vi "GearCollecter_OperatorAssist.vi"(6 "CatchPosition":dbl, 7 "ReturnToCatch":bool, 8 "CarriageReturned":bool, 9 "Manual_Overide":bool, 10 "Start":bool, 11 "Gear_Beam_Break_Sensor_Triggered":bool) -> (0 "Gear_Rail_Position":dbl, 1 "GearChuteExtend":bool, 2 "Catch_Complete?":bool, 3 "Gate_Pos":T1, 4 "Current_State":T2)   [LabVIEW 2016]
uses:
  TypeDefs/GearCollectState_Type.ctl
  TypeDefs/GatePos_Type.ctl
  ArgosLib/Signal Processing/TypeDefs/EdgeDetector_Type.ctl
  ArgosLib/ArgosLib.lvlib
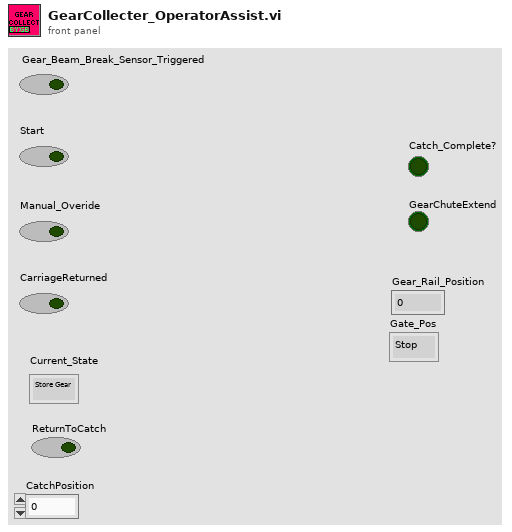
[diagram p1: front panel]
types:
  T1 = typedef "GatePos_Type.ctl" = enum16{"Stop", "Catch", "Clamp", "Open"}
  T2 = typedef "GearCollectState_Type.ctl" = enum16{"Store Gear", "Wait For Gear", "Idle"}
  T3 = typedef "EdgeDetector_Type.ctl" = enum16{"RisingEdge", "FallingEdge", "Both"}
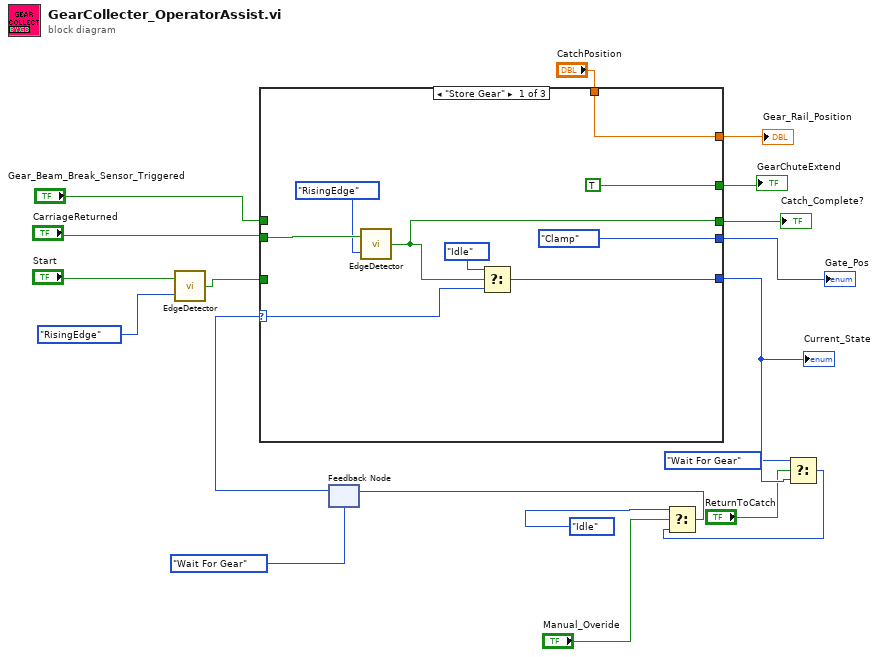
[diagram p0: block diagram]
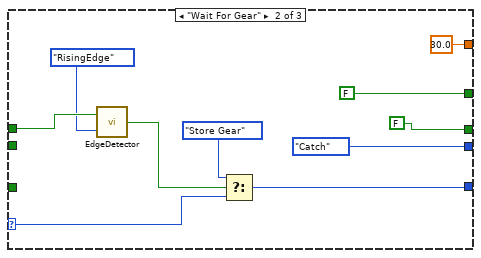
[diagram p2: hidden frame]
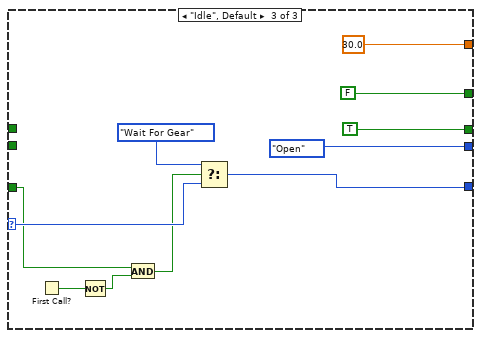
[diagram p3: hidden frame]
diagram:
  n1 = call "EdgeDetector.vi"("DetectorType"=EdgeDetector_Type."RisingEdge", "Input"="Start") -> ("Edge"=w2:bool)
  n2 = feedback #1(GearCollectState_Type."Wait For Gear" ("Gear_Collector_State")) -> (w19:T2)
  n3 = case shown="\"Store Gear\"" w19 {
    selector: w19 -> [w28 w38 w49]
    tunnel: w2 -> [_ _ w39]
    tunnel: [w26 w36 w47] -> w7
    tunnel: "Gear_Beam_Break_Sensor_Triggered" -> [_ w33 _]
    tunnel: "CarriageReturned" -> [w23 _ _]
    tunnel: [GatePos_Type."Clamp" ("Gate_Pos") GatePos_Type."Catch" ("Gate_Pos") GatePos_Type."Open" ("Gate_Pos")] -> w13
    tunnel: [TRUE ("Extend?") FALSE ("Extend?") FALSE ("Extend?")] -> w12
    tunnel: [w21 FALSE ("Extend?") TRUE] -> w10
    tunnel: [w20 30.0 30.0] -> w9
    tunnel: "CatchPosition" -> [w20 _ _]
    frame "Store Gear" {
      n4 = call "EdgeDetector.vi"("DetectorType"=EdgeDetector_Type."RisingEdge", "Input"=w23) -> ("Edge"=w21:bool)
      n5 = Select(t=GearCollectState_Type."Idle", s=w21, f=w28) -> (s? t:f=w26:T2)
    }
    frame "Wait For Gear" {
      n6 = call "EdgeDetector.vi"("DetectorType"=EdgeDetector_Type."RisingEdge", "Input"=w33) -> ("Edge"=w31:bool)
      n7 = Select(t=GearCollectState_Type."Store Gear", s=w31, f=w38) -> (s? t:f=w36:T2)
    }
    frame "Idle", Default {
      n8 = First Call?() -> (First Call?: T/F=w42:bool)
      n9 = Not(x=w42) -> (.not. x?=w43:bool)
      n10 = And(x=w39, y=w43) -> (x .and. y?=w41:bool)
      n11 = Select(t=GearCollectState_Type."Wait For Gear", s=w41, f=w49) -> (s? t:f=w47:T2)
    }
  }
  "GearChuteExtend" <- w12
  "Current_State" <- w7
  "Catch_Complete?" <- w10
  "Gear_Rail_Position" <- w9
  "Gate_Pos" <- w13
  n12 = Select(t=GearCollectState_Type."Wait For Gear", s="ReturnToCatch", f=w7) -> (s? t:f=w8:T2)
  n13 = Select(t=GearCollectState_Type."Idle", s="Manual_Overide", f=w8) -> (s? t:f=w14:T2)
  n14 = feedback-in #1(w14) -> ()
